vi "LoadQ0File.vi"(11 "Q0 external file":path) -> (0 "error out":errorcluster, 3 "FileData":dbl[][](array[numeric]))   [LabVIEW 2025]
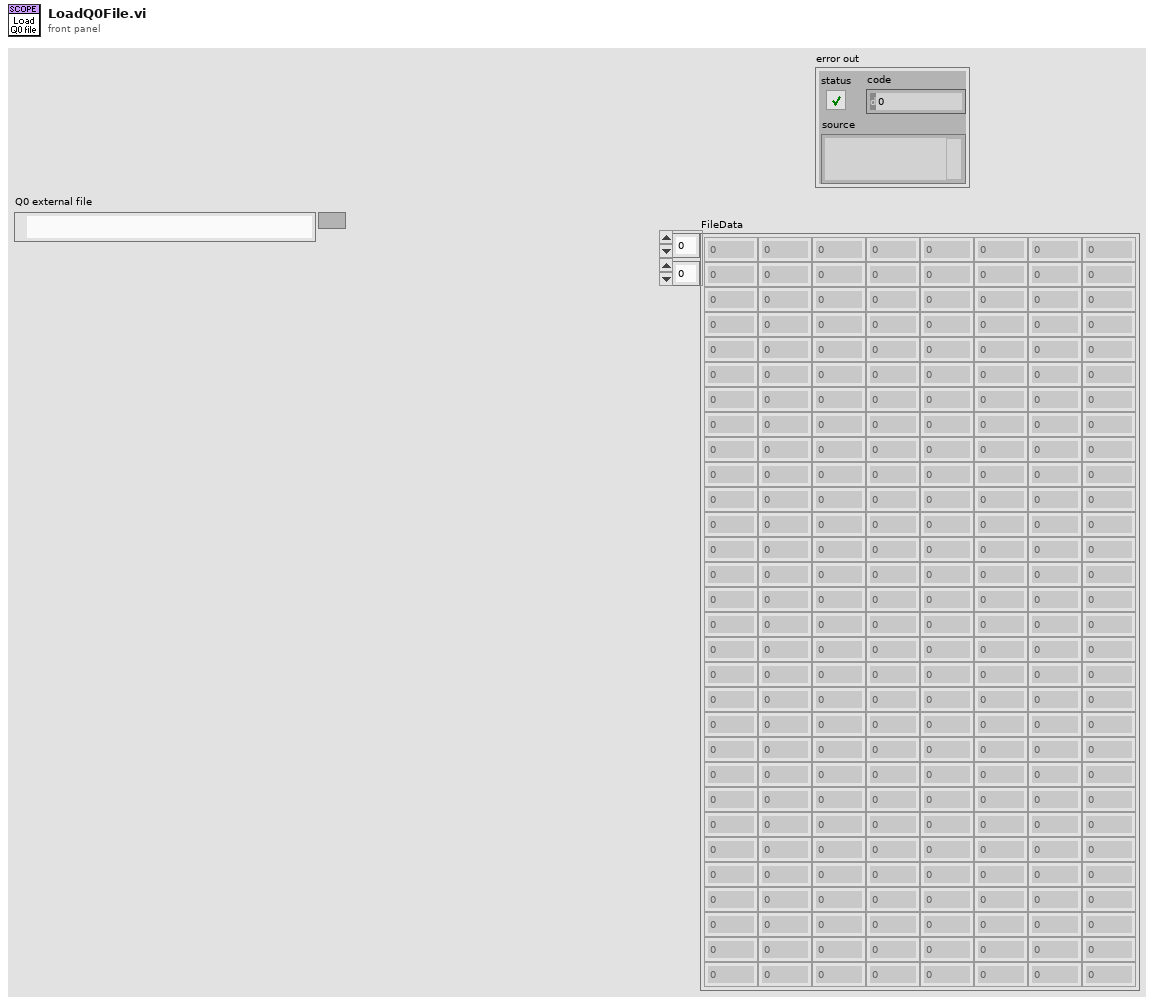
[diagram p1: front panel]
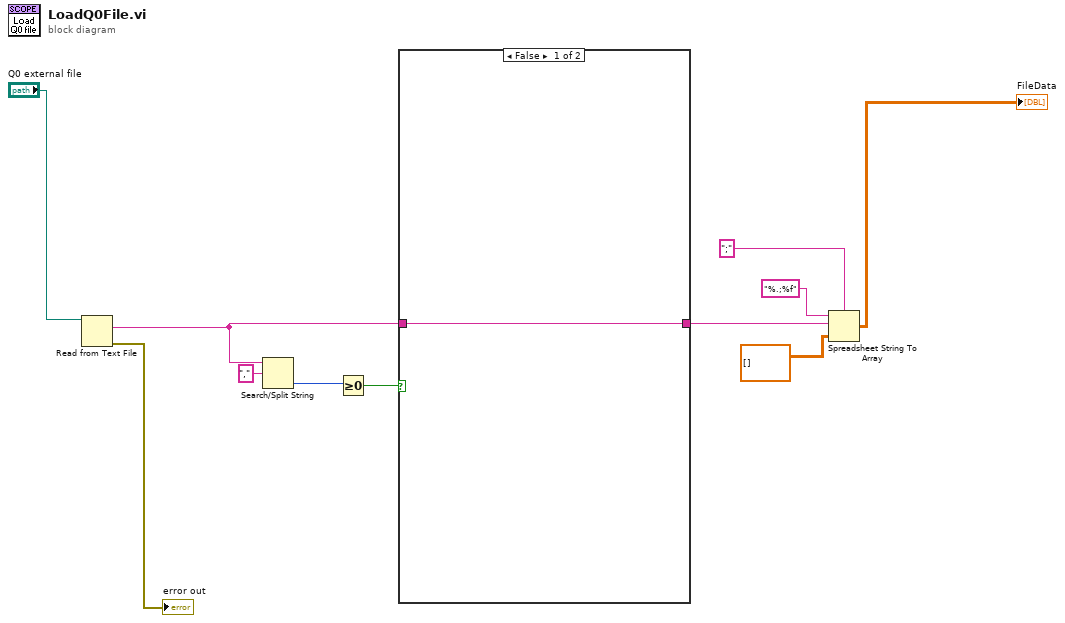
[diagram p0: block diagram]
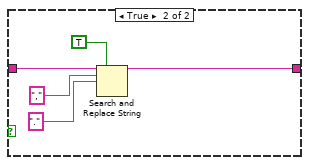
[diagram p2: hidden frame]
diagram:
  n1 = Read from Text File(file (use dialog)="Q0 external file") -> (text=w3:string, error out=→"error out":errorcluster)  [unwired: 3 in, 2 out]
  n2 = Search/Split String(string=w3, search string/char (-)=",") -> (offset of match=w5:i32)  [unwired: 1 in, 2 out]
  n3 = Greater Or Equal To 0?(x=w5) -> (x >= 0?=w4:bool)
  n4 = case shown="False" w4 {
    tunnel: w3 -> [w12 w17]
    tunnel: [w12 w13] -> w2
    frame False {
    }
    frame True {
      n5 = Search and Replace String(replace all?=TRUE ("replace all? (F)"), input string=w17, search string=",", replace string="." ("replace string (\"\")")) -> (result string=w13:string)  [unwired: 4 in, 3 out]
    }
  }
  n6 = Spreadsheet String To Array(delimiter (Tab)=";" ("delimiter (\\t)"), format string="%.;%f", spreadsheet string=w2, array type (2D Dbl)=dbl[][] [] ("type (empty)")) -> (array=→"FileData":dbl[][])
